vi "Panel.vi"(11 "AppDetailPanel in":refnum<class "AppDetailPanel.lvclass">) -> ()   [LabVIEW 2020, in "PicoG-App.lvlib" / "AppDetailPanel.lvclass"]
uses:
  AppDetailPanel.lvclass
  C:/Program Files (x86)/National Instruments/LabVIEW 2020/vi.lib/IlluminatedG/IG OOPanel/OOPanel/Panel/Panel.lvclass
  Device/Device.lvclass
  <vilib>/IlluminatedG/IG OOPanel/OOPanel/Panel/Basic UI State.ctl
  AppDetailPanel.lvclass/AppDetailPanel.ctl
  Builds/picoG/ppl/PicoG-Core.lvlibp/PicoG-Processor/PicoG-Core/Platform/Platform.lvclass
  <vilib>/IlluminatedG/IG OOPanel/OOPanel/Panel/Panel.lvclass
  <vilib>/IlluminatedG/IG OOPanel/OOPanel/OOPanel.lvlib
  ViaApp/ViaApp.lvclass
panel:
  out "Devices":refnum<class "Device.lvclass">[](array[class])
  in  "Remove":bool
  out "Name":string
  in  "Explore":bool
  out "App Path":path
  in  "Preview":bool
  in  "Deploy":bool
  in  "Device":string(combo)="<No Configured Devices>"
  out "Source":string
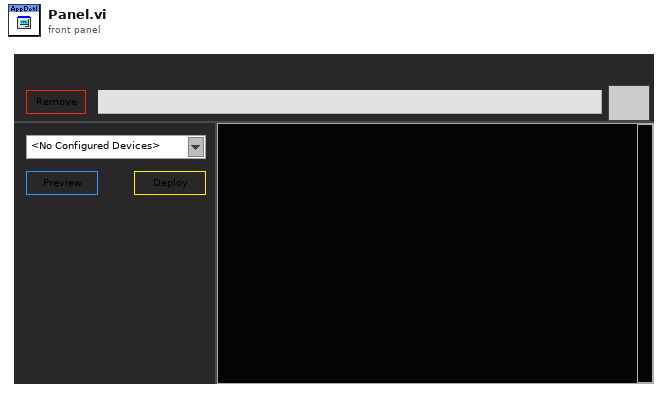
[diagram p1: front panel]
types:
  T1 = typedef "OOPanel.lvlib/Panel.lvclass/Basic UI State.ctl" = enum16{"Init", "Run", "Close"}
  T2 = typedef "PicoG-App.lvlib/AppDetailPanel.lvclass/Inbound Events.ctl" = cluster{"App Updated":refnum<user-event>, "Device List (Ext)":refnum<user-event>}
  T3 = typedef "OOPanel.lvlib/Panel.lvclass/Panel Events.ctl" = cluster{"Visbility":refnum<user-event>, "Close":refnum<user-event>}
  T4 = typedef "PicoG-App.lvlib/AppDetailPanel.lvclass/Ref Data.ctl" = cluster{"App":refnum<class "ViaApp.lvclass">}
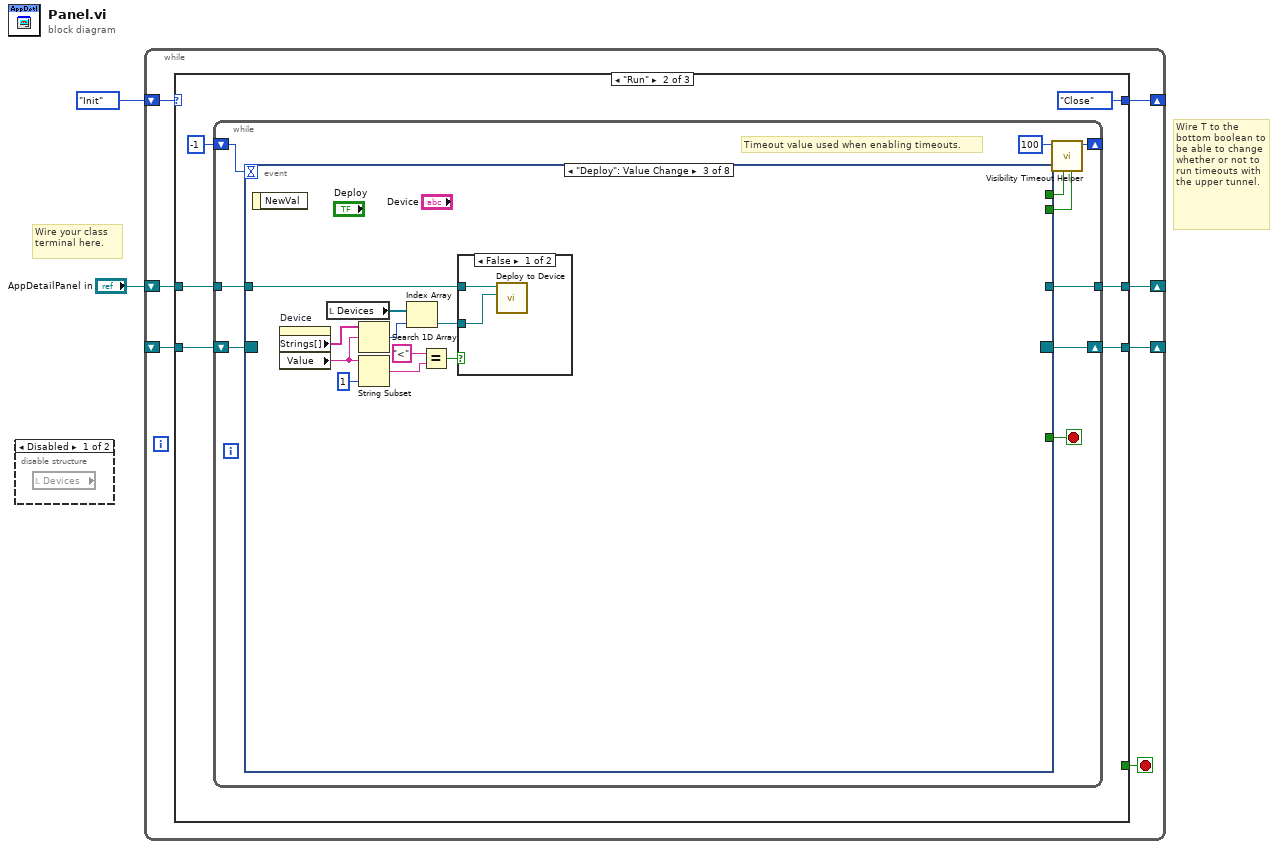
[diagram p0: block diagram]
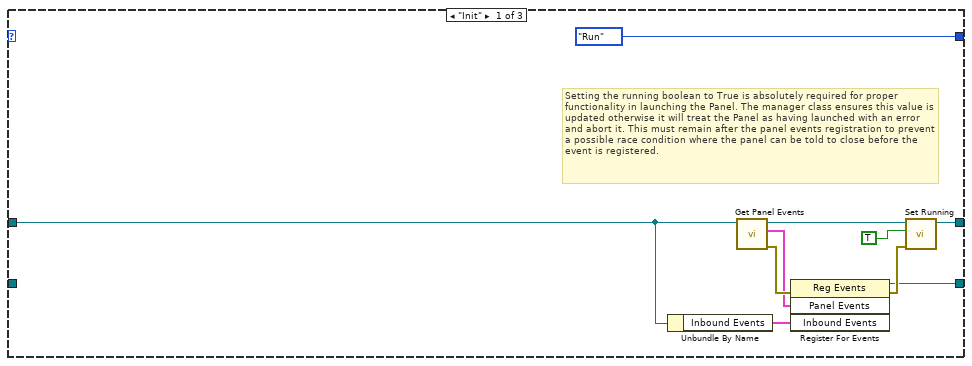
[diagram p3: hidden frame]
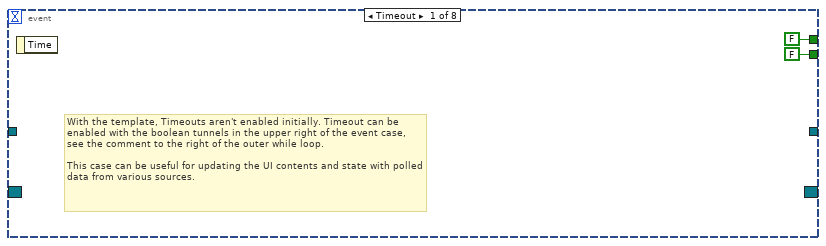
[diagram p4: hidden frame]
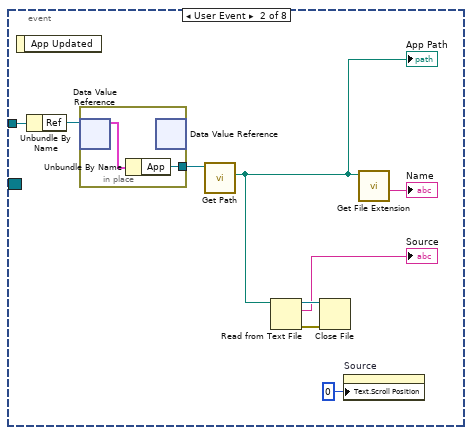
[diagram p5: hidden frame]
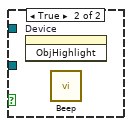
[diagram p6: hidden frame]
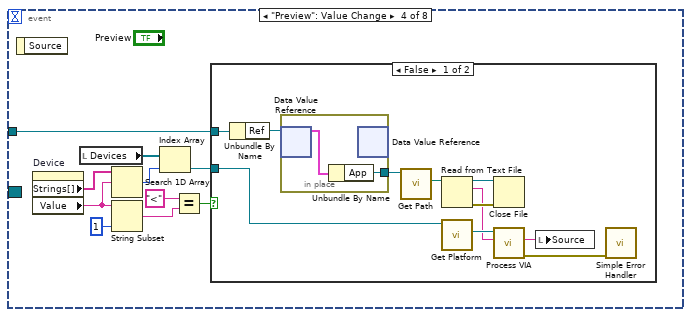
[diagram p7: hidden frame]
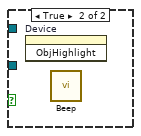
[diagram p8: hidden frame]
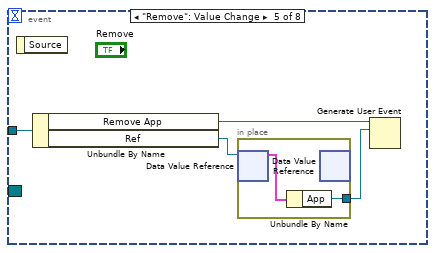
[diagram p9: hidden frame]
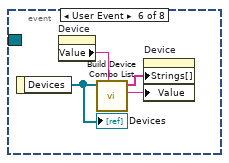
[diagram p10: hidden frame]
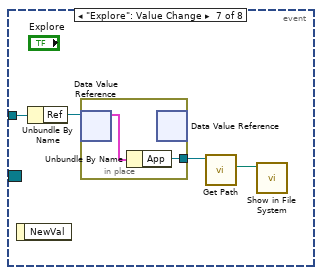
[diagram p11: hidden frame]
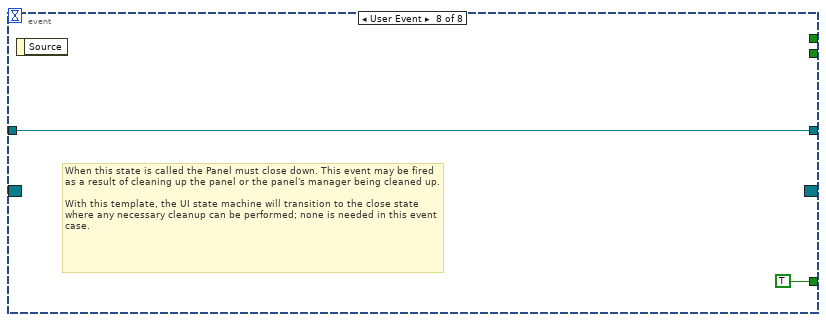
[diagram p12: hidden frame]
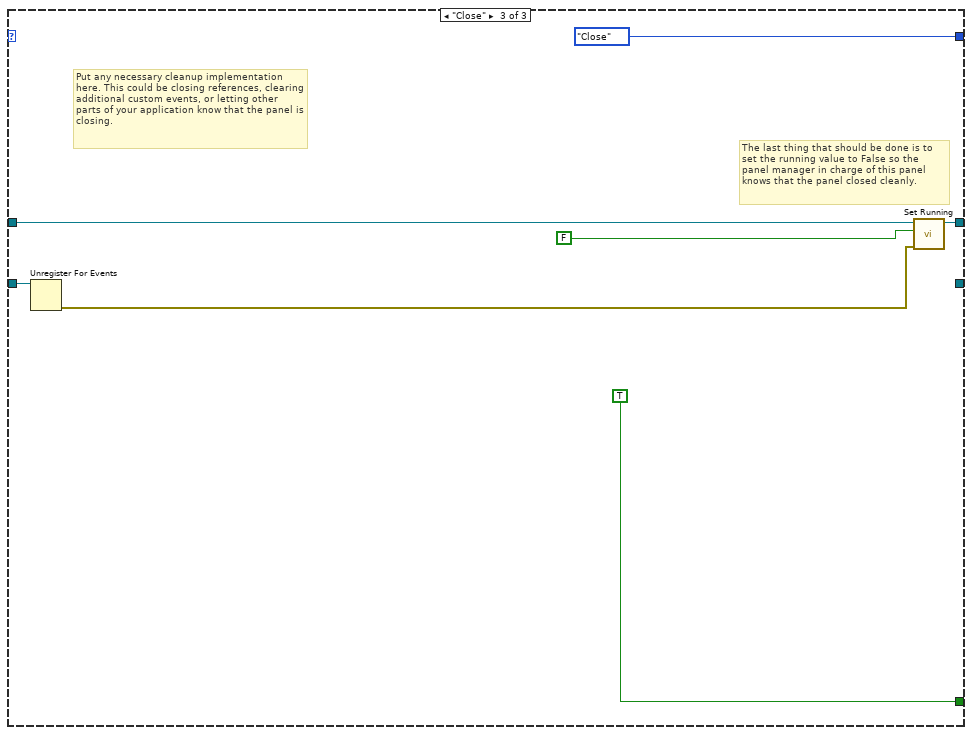
[diagram p13: hidden frame]
diagram:
  # "Wire T to the bottom boolean to be able to change whether or not to run timeouts with the upper tunnel."
  # "Wire your class terminal here."
  n1 = disable-structure shown="Disabled" {
    frame Disabled {
      n2 = local read "Devices"() -> ()  [unwired: 1 out]
    }
    frame Enabled {
    }
  }
  n3 = while {
    shift-right: [w8] -> _
    shift-left: _ -> [w9]
    shift-right: [w6] -> _
    shift-left: Basic_UI_State."Init" ("Basic UI State") -> [w7]
    shift-right: [w4] -> _
    shift-left: "AppDetailPanel in" -> [w3]
    stop <- w5 stop-if-true
    n4 = case shown="\"Run\"" w7 {
      tunnel: w9 -> [_ w25 w104]
      tunnel: [w13 w23 _] -> w8
      tunnel: [Basic_UI_State."Run" ("Basic UI State") Basic_UI_State."Close" ("Basic UI State") Basic_UI_State."Close" ("Basic UI State")] -> w6
      tunnel: [_ _ TRUE] -> w5
      tunnel: [w12 w20 w102] -> w4
      tunnel: w3 -> [w11 w21 w103]
      frame "Init" {
        # "Setting the running boolean to True is absolutely required for proper functionality in launching the Panel. The manager class ensures this value is updated otherwise it will treat the Panel as having launched with an error and abort it. This must remain after the panel events registration to prevent a possible race condition where the panel can be told to close before the event is registered."
        n5 = Unbundle By Name(w11) -> ("Inbound Events"=w10:T2)
        n6 = call <vilib>:"Get Panel Events.vi"("Panel in"=w11) -> ("error out"=w19:errorcluster, "Panel Events"=w15:T3, "Panel out"=w16:refnum<class "AppDetailPanel.lvclass">)  [unwired: 8 in]
        n7 = register-events(error in=w19, w15, w10) -> (reference out=w13:refnum<event-registration>, error out=w17:errorcluster)  [unwired: 1 in]
        n8 = call <vilib>:"Set Running.vi"("error in (no error)"=w17, "Running"=TRUE, "Panel in"=w16) -> ("Panel out"=w12:refnum<class "AppDetailPanel.lvclass">)  [unwired: 7 in, 1 out]
      }
      frame "Run" {
        n9 = while {
          shift-right: [w31] -> w23
          shift-left: w25 -> [w32]
          shift-right: [w34] -> _
          shift-left: -1 ("Timeout") -> [w33]
          tunnel: w21 -> [w27]
          tunnel: [w26] -> w20
          stop <- w28 stop-if-true
          # "Timeout value used when enabling timeouts."
          n10 = event shown="[2] \"Deploy\": Value Change" {
            selector: w32 -> [_ _ _ _ _ _ _ _]
            dyn-events: [_ _ _ _ _ _ _ _] -> w31
            timeout: w33 -> [_ _ _ _ _ _ _ _]
            tunnel: [FALSE _ _ _ _ _ _ _] -> w30
            tunnel: [FALSE _ _ _ _ _ _ _] -> w29
            tunnel: [_ _ _ _ _ _ _ TRUE] -> w28
            tunnel: w27 -> [_ w45 w54 w61 w86 _ w95 w100]
            tunnel: [_ _ _ _ _ _ _ w100] -> w26
            event Timeout {
              # "With the template, Timeouts aren't enabled initially. Timeout can be enabled with the boolean tunnels in the upper right of the event case, see the comment to the right of the outer while loop.\n\nThis case can be useful for updating the UI contents and state with polled data from various sources."
              n11 = event-data() -> ()  [unwired: 1 in, 1 out]
            }
            event User Event {
              n12 = event-data() -> ()  [unwired: 1 in, 1 out]
              n13 = Unbundle By Name(w45) -> ("Ref"=w46:refnum<data-value>)
              n14 = in-place {
                in-place-border: [w47] -> w44
                n15 = in-place-dvr #1(w46) -> (w48:T4)  [unwired: 1 out]
                n16 = Unbundle By Name(w48) -> ("App"=w47:refnum<class "ViaApp.lvclass">)
                n17 = in-place-dvr #1() -> ()  [unwired: 1 in, 2 out]
              }
              n18 = call "Get Path.vi"("ViaApp in"=w44) -> ("Path"=w42:path)  [unwired: 8 in, 2 out]
              "App Path" <- w42
              n19 = Read from Text File(file (use dialog)=w42) -> (refnum out=w41:refnum<file>, text=→"Source":string, error out=w40:errorcluster)  [unwired: 3 in, 1 out]
              n20 = Close File(refnum=w41, error in=w40) -> ()  [unwired: 2 out]
              n21 = property on="Source" class="Str"("Text.Scroll Position"=u32 0) -> ()  [unwired: 2 in, 2 out]
              n22 = call <vilib>:"Get File Extension.vi"("file"=w42) -> ("filename without extension"=→"Name":string)  [unwired: 6 in, 4 out]
            }
            event "Deploy": Value Change {
              n23 = event-data() -> ()  [unwired: 1 in, 1 out]
              n24 = property on="Device" class="CmbBox"() -> ("Strings[]"=w52:string[], "Value"=w53:string)  [unwired: 2 in, 2 out]
              n25 = local read "Devices"() -> (w51:refnum<class "Device.lvclass">[])
              n26 = Search 1D Array(1D array=w52, element=w53) -> (index of element=w50:i32)  [unwired: 1 in]
              n27 = String Subset(string=w53, length (rest)=1 ("length (rest)")) -> (substring=w57:string)  [unwired: 1 in]
              n28 = Index Array(array=w51, index=w50) -> (element=w49:refnum<class "Device.lvclass">)
              n29 = Equal?(x="<" ("regular expression"), y=w57) -> (x = y?=w55:bool)
              n30 = case shown="False" w55 {
                tunnel: w54 -> [w60 _]
                tunnel: w49 -> [w59 _]
                frame False {
                  n31 = call "Deploy to Device.vi"("Device"=w59, "AppDetailPanel in"=w60) -> ()  [unwired: 8 in, 2 out]
                }
                frame True {
                  n32 = invoke on="Device" class="CmbBox" method="ObjHighlight"() -> ()  [unwired: 3 in, 3 out]
                  n33 = call <vilib>:"Beep.vi"() -> ()  [unwired: 12 in]
                }
              }
            }
            event "Preview": Value Change {
              n34 = event-data() -> ()  [unwired: 1 in, 1 out]
              n35 = property on="Device" class="CmbBox"() -> ("Strings[]"=w67:string[], "Value"=w68:string)  [unwired: 2 in, 2 out]
              n36 = local read "Devices"() -> (w66:refnum<class "Device.lvclass">[])
              n37 = Search 1D Array(1D array=w67, element=w68) -> (index of element=w65:i32)  [unwired: 1 in]
              n38 = String Subset(string=w68, length (rest)=1 ("length (rest)")) -> (substring=w70:string)  [unwired: 1 in]
              n39 = Index Array(array=w66, index=w65) -> (element=w64:refnum<class "Device.lvclass">)
              n40 = Equal?(x="<" ("regular expression"), y=w70) -> (x = y?=w69:bool)
              n41 = case shown="False" w69 {
                tunnel: w61 -> [w75 _]
                tunnel: w64 -> [w73 _]
                frame False {
                  n42 = Unbundle By Name(w75) -> ("Ref"=w76:refnum<data-value>)
                  n43 = in-place {
                    in-place-border: [w82] -> w74
                    n44 = in-place-dvr #2(w76) -> (w83:T4)  [unwired: 1 out]
                    n45 = Unbundle By Name(w83) -> ("App"=w82:refnum<class "ViaApp.lvclass">)
                    n46 = in-place-dvr #2() -> ()  [unwired: 1 in, 2 out]
                  }
                  n47 = call "Get Path.vi"("ViaApp in"=w74) -> ("Path"=w77:path)  [unwired: 8 in, 2 out]
                  n48 = Read from Text File(file (use dialog)=w77) -> (refnum out=w80:refnum<file>, text=w78:string, error out=w79:errorcluster)  [unwired: 3 in, 1 out]
                  n49 = call "Get Platform.vi"("Device in"=w73) -> ("Platform"=w81:refnum<class "Platform.lvclass">)  [unwired: 8 in, 2 out]
                  n50 = Close File(refnum=w80, error in=w79) -> ()  [unwired: 2 out]
                  n51 = call-dynamic "Process VIA.vi"("Raw VIA"=w78, "DeployTarget in"=w81) -> ("error out"=w72:errorcluster, "VIA"=w71:string)  [unwired: 7 in, 1 out]
                  n52 = local write "Source"(w71) -> ()
                  n53 = call <vilib>:"Simple Error Handler.vi"("error in (no error)"=w72) -> ()  [unwired: 4 in, 5 out]
                }
                frame True {
                  n54 = invoke on="Device" class="CmbBox" method="ObjHighlight"() -> ()  [unwired: 3 in, 3 out]
                  n55 = call <vilib>:"Beep.vi"() -> ()  [unwired: 12 in]
                }
              }
            }
            event "Remove": Value Change {
              n56 = event-data() -> ()  [unwired: 1 in, 1 out]
              n57 = Unbundle By Name(w86) -> ("Remove App"=w85:refnum<user-event>, "Ref"=w87:refnum<data-value>)
              n58 = in-place {
                in-place-border: [w88] -> w84
                n59 = in-place-dvr #3(w87) -> (w89:T4)  [unwired: 1 out]
                n60 = Unbundle By Name(w89) -> ("App"=w88:refnum<class "ViaApp.lvclass">)
                n61 = in-place-dvr #3() -> ()  [unwired: 1 in, 2 out]
              }
              n62 = Generate User Event(user event=w85, event data cluster=w84) -> ()  [unwired: 2 in, 2 out]
            }
            event User Event {
              n63 = event-data() -> ("Devices"=w93:refnum<class "Device.lvclass">[])  [unwired: 1 in]
              "Devices" <- w93
              n64 = property on="Device" class="CmbBox"() -> ("Value"=w92:string)  [unwired: 2 in, 2 out]
              n65 = call "Build Device Combo List.vi"("Previous Value"=w92, "Devices"=w93) -> ("Value"=w90:string, "Strings"=w91:string[])  [unwired: 8 in]
              n66 = property on="Device" class="CmbBox"("Strings[]"=w91, "Value"=w90) -> ()  [unwired: 2 in, 2 out]
            }
            event "Explore": Value Change {
              n67 = event-data() -> ()  [unwired: 1 in, 1 out]
              n68 = Unbundle By Name(w95) -> ("Ref"=w97:refnum<data-value>)
              n69 = in-place {
                in-place-border: [w98] -> w96
                n70 = in-place-dvr #4(w97) -> (w99:T4)  [unwired: 1 out]
                n71 = Unbundle By Name(w99) -> ("App"=w98:refnum<class "ViaApp.lvclass">)
                n72 = in-place-dvr #4() -> ()  [unwired: 1 in, 2 out]
              }
              n73 = call "Get Path.vi"("ViaApp in"=w96) -> ("Path"=w94:path)  [unwired: 8 in, 2 out]
              n74 = call <vilib>:"Show in File System.vi"("file or directory path"=w94) -> ()  [unwired: 10 in, 1 out]
            }
            event User Event {
              # "When this state is called the Panel must close down. This event may be fired as a result of cleaning up the panel or the panel's manager being cleaned up.\n\nWith this template, the UI state machine will transition to the close state where any necessary cleanup can be performed; none is needed in this event case."
              n75 = event-data() -> ()  [unwired: 1 in, 1 out]
            }
          }
          n76 = call <vilib>:"Visibility Timeout Helper.vi"("Update?"=w29, "Use Timeout?"=w30, "Visible Timeout mS"=100) -> ("Timeout"=w34:i32)  [unwired: 8 in]
        }
      }
      frame "Close" {
        # "Put any necessary cleanup implementation here. This could be closing references, clearing additional custom events, or letting other parts of your application know that the panel is closing."
        # "The last thing that should be done is to set the running value to False so the panel manager in charge of this panel knows that the panel closed cleanly."
        n77 = Unregister For Events(event registration refnum=w104) -> (error out=w106:errorcluster)  [unwired: 1 in]
        n78 = call <vilib>:"Set Running.vi"("error in (no error)"=w106, "Running"=FALSE, "Panel in"=w103) -> ("Panel out"=w102:refnum<class "AppDetailPanel.lvclass">)  [unwired: 7 in, 1 out]
      }
    }
  }
